vi "RemoveChildFromNode.vi"(8 "error in":errorcluster, 10 "removed child":T1, 11 "Engine Parent Editor Node in":refnum<class "Engine Parent Editor Node.lvclass">) -> (0 "error out":errorcluster, 3 "Engine Parent Editor Node out":refnum<class "Engine Parent Editor Node.lvclass">)   [LabVIEW 2014, in "PL Framework Configuration Tool.lvlib" / "Engine Parent Editor Node.lvclass"]
doc: "Remove module from the target engine.\n\nRemoving the module will delete all channels mapped to that module."
uses:
  Engine Parent Editor Node.lvclass
  <vilib>/NI/Configuration Framework/Node/NodeRef.ctl
  <vilib>/NI/Configuration Framework/Node/NISE_CEF_Node.lvclass
  <vilib>/NI/Configuration Framework/serializable node/NISE_CEF_serializable node.lvclass
  Targets/Targets.lvclass
  <vilib>/NI/Configuration Framework/Node/NISE_CEF_Node.lvclass/NISE_CEF_Node.ctl
  <vilib>/NI/Configuration Framework/serializable configuration/NISE_CEF_serializable configuration.lvclass/NISE_CEF_serializable configuration.ctl
  Targets/Targets.lvclass/Targets.ctl
  Targets/Read Configuration Class Name.vi
  Targets/Write Configuration Class Name.vi
  <vilib>/Utility/LVClass/Get LV Class Name.vi
  <vilib>/NI/Configuration Framework/error generator/NISE_error generator.vi
  read engine configuration.vi
  write engine configuration.vi
  <vilib>/NI/Configuration Framework/serializable configuration/NISE_CEF_serializable configuration.lvclass
  <vilib>/NI/Module Execution Interface/Engine Configuration/engine configuration.lvclass
  TBM Configuration Node/TBM Configuration Node.lvclass
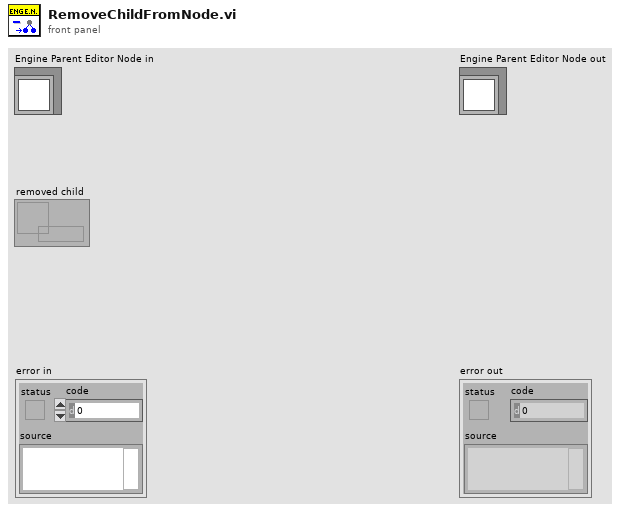
[diagram p1: front panel]
types:
  T1 = typedef "NISE_CEF_Node.lvclass/NodeRef.ctl" = refnum<data-value>
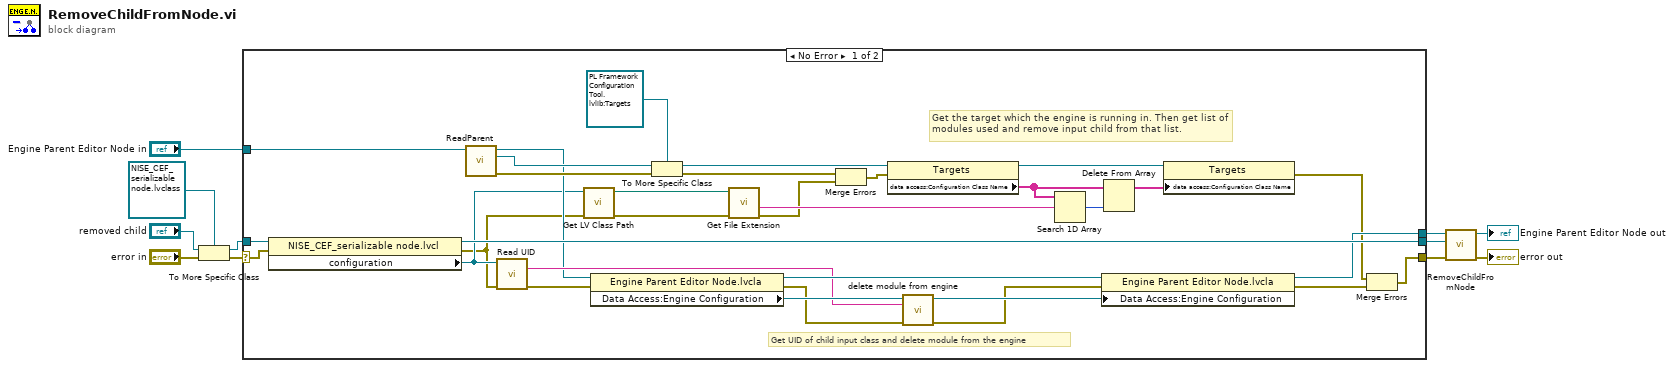
[diagram p0: block diagram]
diagram:
  n1 = To More Specific Class(target class=refnum<data-value> refnum, reference="removed child", error in="error in") -> (specific class reference=w10:refnum<data-value>, error out=w8:errorcluster)
  n2 = case shown="No Error" w8 {
    selector: w8 -> [w41 w44]
    tunnel: [w14 w44] -> w7
    tunnel: [w43 w45] -> w11
    tunnel: w10 -> [w42 w45]
    tunnel: "Engine Parent Editor Node in" -> [w24 w46]
    tunnel: [w39 w46] -> w6
    frame No Error {
      # "Get the target which the engine is running in. Then get list of modules used and remove input child from that list."
      # "Get UID of child input class and delete module from the engine"
      n3 = property class="NISE_CEF_serializable node.lvcl"(reference=w42, error in=w41) -> (reference out=w43:refnum<data-value>, error out=w13:errorcluster, "configuration"=w22:refnum<class "NISE_CEF_serializable configuration.lvclass">)
      n4 = call <vilib>:"ReadParent.vi"("node in"=w24) -> ("error out"=w31:errorcluster, "parent"=w29:T1, "node out"=w23:refnum<class "Engine Parent Editor Node.lvclass">)  [unwired: 8 in]
      n5 = call <vilib>:"Read UID.vi"("error in"=w13, "configuration in"=w22) -> ("error out"=w40:errorcluster, "instance id"=w33:string)  [unwired: 7 in, 1 out]
      n6 = call <vilib>:"Get LV Class Path.vi"("error in (no error)"=w13, "object"=w22) -> ("error out"=w21:errorcluster, "class path"=w27:path)  [unwired: 8 in]
      n7 = property class="Engine Parent Editor Node.lvcla"(reference=w23, error in=w40) -> (reference out=w38:refnum<class "Engine Parent Editor Node.lvclass">, error out=w34:errorcluster, "Data Access:Engine Configuration"=w37:refnum<class "engine configuration.lvclass">)
      n8 = To More Specific Class(target class=refnum<data-value> refnum, reference=w29, error in=w31) -> (specific class reference=w30:refnum<data-value>, error out=w26:errorcluster)
      n9 = call <vilib>:"Get File Extension.vi"("error in (no error)"=w21, "file"=w27) -> ("error out"=w17:errorcluster, "filename without extension"=w18:string)  [unwired: 6 in, 2 out]
      n10 = Merge Errors(w26, w17) -> (w25:errorcluster)
      n11 = property class="Targets"(reference=w30, error in=w25) -> (reference out=w28:refnum<data-value>, "data access:Configuration Class Name"=w20:string[])  [unwired: 1 out]
      n12 = call-dynamic "delete module from engine.vi"("error in"=w34, "module ID"=w33, "engine configuration in"=w37) -> ("error out"=w35:errorcluster, "engine configuration out"=w36:refnum<class "engine configuration.lvclass">)  [unwired: 7 in]
      n13 = Search 1D Array(1D array=w20, element=w18) -> (index of element=w12:i32)  [unwired: 1 in]
      n14 = property class="Engine Parent Editor Node.lvcla"(reference=w38, error in=w35, "Data Access:Engine Configuration"=w36) -> (reference out=w39:refnum<class "Engine Parent Editor Node.lvclass">, error out=w15:errorcluster)
      n15 = Delete From Array(array=w20, index=w12) -> (array with subset deleted=w19:string[])  [unwired: 1 in, 1 out]
      n16 = property class="Targets"(reference=w28, "data access:Configuration Class Name"=w19) -> (error out=w16:errorcluster)  [unwired: 1 in, 1 out]
      n17 = Merge Errors(w16, w15) -> (w14:errorcluster)
    }
    frame Error {
    }
  }
  n18 = call-parent "RemoveChildFromNode.vi"("error in"=w7, "removed child"=w11, "NISE_CEF_Node in"=w6) -> ("error out"=→"error out":errorcluster, "NISE_CEF_Node out"=→"Engine Parent Editor Node out":refnum<class "Engine Parent Editor Node.lvclass">)  [unwired: 7 in]
